vi "Single Axis motor_Z(SubVI).vi"(0 "State=1, I":dbl, 1 "Motor=0, I":i32, 2 "Position=0, I":dbl, 3 "User Input":dbl, 4 "Motor Input":dbl, 5 "Backward":bool, 6 "Forward":bool, 7 "Step diff":dbl, 9 "Motor input_L":refnum<vi>, 11 "User input_L":refnum<vi>, 13 "Step diff_L":refnum<vi>) -> (15 "right":bool, 17 "down":bool, 18 "State Chart":i32(graph), 19 "Motor State":dbl, 20 "State=1, O":dbl, 21 "Motor=0, O":i32, 22 "Position=0, O":dbl, 23 "Real Output":dbl, 24 "Motor Position":dbl, 25 "up":bool, 26 "left":bool, 27 "Moving":bool)   [LabVIEW 2018]
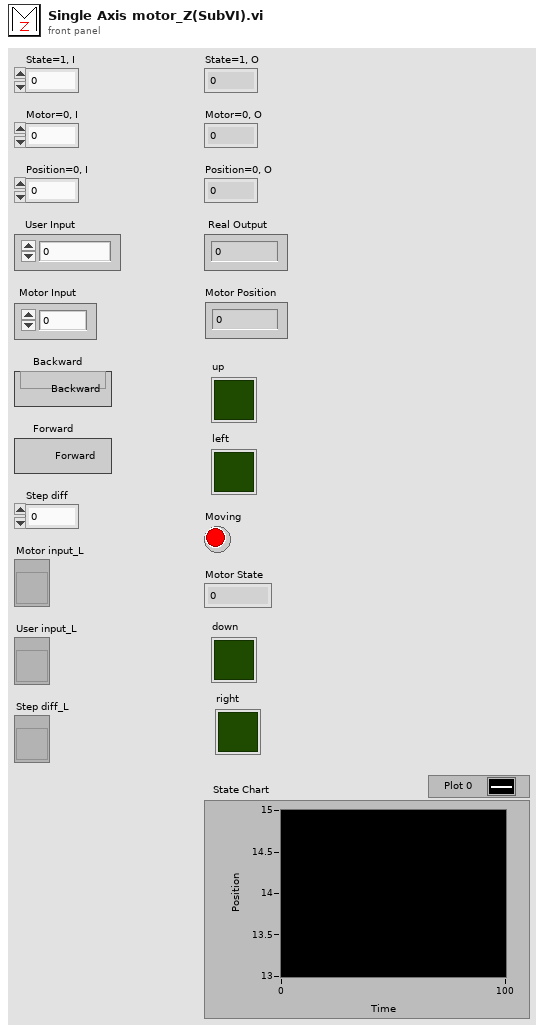
[diagram p1: front panel]
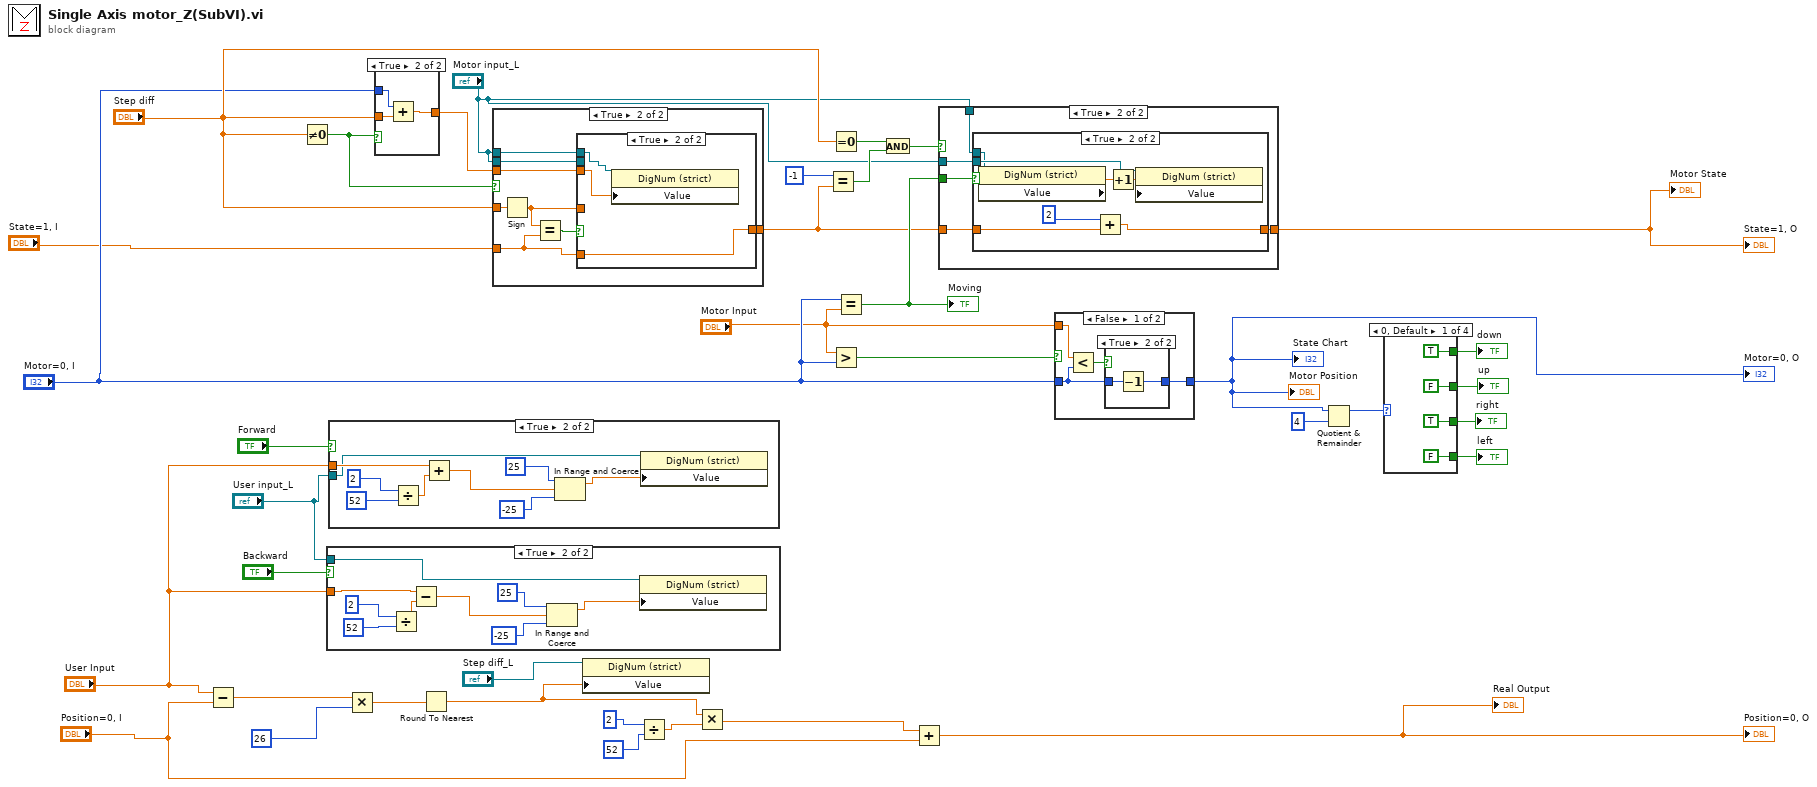
[diagram p0: block diagram]
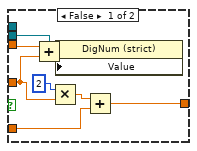
[diagram p7: hidden frame]
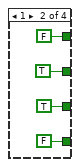
[diagram p8: hidden frame]
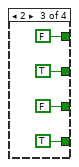
[diagram p9: hidden frame]
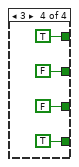
[diagram p10: hidden frame]
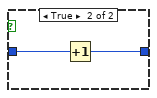
[diagram p12: hidden frame]
diagram:
  n1 = Subtract(x="User Input", y="Position=0, I") -> (x-y=w15:dbl)
  n2 = Not Equal To 0?(x="Step diff") -> (x != 0?=w9:bool)
  n3 = case shown="True" "Backward" {
    tunnel: "User Input" -> [_ w43]
    tunnel: "User input_L" -> [_ w42]
    frame False {
    }
    frame True {
      n4 = Divide(x=2, y=52) -> (x/y=w44:dbl)
      n5 = Subtract(x=w43, y=w44) -> (x-y=w39:dbl)
      n6 = In Range and Coerce(upper limit=25, x=w39, lower limit=-25) -> (coerced(x)=w38:dbl)  [unwired: 1 out]
      n7 = property class="DigNum (strict)"(reference=w42, "Value"=w38) -> ()  [unwired: 1 in, 2 out]
    }
  }
  n8 = case shown="True" "Forward" {
    tunnel: "User Input" -> [_ w52]
    tunnel: "User input_L" -> [_ w51]
    frame False {
    }
    frame True {
      n9 = Divide(x=2, y=52) -> (x/y=w53:dbl)
      n10 = Add(x=w52, y=w53) -> (x+y=w48:dbl)
      n11 = In Range and Coerce(upper limit=25, x=w48, lower limit=-25) -> (coerced(x)=w47:dbl)  [unwired: 1 out]
      n12 = property class="DigNum (strict)"(reference=w51, "Value"=w47) -> ()  [unwired: 1 in, 2 out]
    }
  }
  n13 = Multiply(x=w15, y=26) -> (x*y=w16:dbl)
  n14 = case shown="True" w9 {
    tunnel: "Motor=0, I" -> [_ w59]
    tunnel: "Step diff" -> [w56 w58]
    tunnel: [w56 w57] -> w10
    frame False {
    }
    frame True {
      n15 = Add(x=w59, y=w58) -> (x+y=w57:dbl)
    }
  }
  n16 = Round To Nearest(number=w16) -> (nearest integer value=w20:dbl)
  n17 = case shown="True" w9 {
    tunnel: [w60 w67] -> w26
    tunnel: "State=1, I" -> [w60 w66]
    tunnel: "Step diff" -> [_ w64]
    tunnel: w10 -> [_ w63]
    tunnel: "Motor input_L" -> [_ w62]
    tunnel: "Motor input_L" -> [_ w61]
    frame False {
    }
    frame True {
      n18 = Sign(1:w64) -> (0:w65:dbl)
      n19 = Equal?(x=w65, y=w66) -> (x = y?=w68:bool)
      n20 = case shown="True" w68 {
        tunnel: w65 -> [w70 _]
        tunnel: [w75 w79] -> w67
        tunnel: w66 -> [w73 w79]
        tunnel: w63 -> [w72 w78]
        tunnel: w62 -> [w69 _]
        tunnel: w61 -> [_ w77]
        frame False {
          n21 = Add(x=w72, y=w70) -> (x+y=w74:dbl)
          n22 = Multiply(x=2, y=w70) -> (x*y=w71:dbl)
          n23 = property class="DigNum (strict)"(reference=w69, "Value"=w74) -> ()  [unwired: 1 in, 2 out]
          n24 = Add(x=w71, y=w73) -> (x+y=w75:dbl)
        }
        frame True {
          n25 = property class="DigNum (strict)"(reference=w77, "Value"=w78) -> ()  [unwired: 1 in, 2 out]
        }
      }
    }
  }
  n26 = property class="DigNum (strict)"(reference="Step diff_L", "Value"=w20) -> ()  [unwired: 1 in, 2 out]
  n27 = Divide(x=2, y=52) -> (x/y=w19:dbl)
  n28 = Multiply(x=w20, y=w19) -> (x*y=w6:dbl)
  n29 = Equal?(x=-1, y=w26) -> (x = y?=w25:bool)
  n30 = Equal To 0?(x="Step diff") -> (x = 0?=w24:bool)
  n31 = Greater?(x="Motor Input", y="Motor=0, I") -> (0:w8:bool)
  n32 = Equal?(x="Motor=0, I", y="Motor Input") -> (x = y?=w36:bool)
  "Moving" <- w36
  n33 = And(x=w24, y=w25) -> (x .and. y?=w23:bool)
  n34 = Add(x=w6, y="Position=0, I") -> (x+y=→"Real Output" →"Position=0, O":dbl)
  n35 = case shown="True" w23 {
    tunnel: w26 -> [w80 w84]
    tunnel: [w80 w85] -> w22
    tunnel: w36 -> [_ w83]
    tunnel: "Motor input_L" -> [_ w82]
    tunnel: "Motor input_L" -> [_ w81]
    frame False {
    }
    frame True {
      n36 = case shown="True" w83 {
        tunnel: [w86 w91] -> w85
        tunnel: w84 -> [w86 w92]
        tunnel: w82 -> [_ w88]
        tunnel: w81 -> [_ w87]
        frame False {
        }
        frame True {
          n37 = property class="DigNum (strict)"(reference=w87) -> ("Value"=w89:dbl)  [unwired: 1 in, 2 out]
          n38 = Add(x=2, y=w92) -> (x+y=w91:dbl)
          n39 = Increment(x=w89) -> (x+1=w90:dbl)
          n40 = property class="DigNum (strict)"(reference=w88, "Value"=w90) -> ()  [unwired: 1 in, 2 out]
        }
      }
    }
  }
  "Motor State" <- w22
  "State=1, O" <- w22
  n41 = case shown="False" w8 {
    tunnel: "Motor=0, I" -> [w95 w102]
    tunnel: [w94 w101] -> w21
    tunnel: "Motor Input" -> [w97 _]
    frame False {
      n42 = Less?(x=w97, y=w95) -> (x < y?=w96:bool)
      n43 = case shown="True" w96 {
        tunnel: w95 -> [w98 w100]
        tunnel: [w98 w99] -> w94
        frame False {
        }
        frame True {
          n44 = Decrement(x=w100) -> (x-1=w99:i32)
        }
      }
    }
    frame True {
      n45 = Increment(x=w102) -> (x+1=w101:i32)
    }
  }
  "State Chart" <- w21
  "Motor Position" <- w21
  "Motor=0, O" <- w21
  n46 = Quotient & Remainder(x=w21, y=4) -> (x-y*floor(x/y)=w28:i32)  [unwired: 1 out]
  n47 = case shown="0, Default" w28 {
    tunnel: [FALSE FALSE TRUE TRUE] -> w32
    tunnel: [TRUE TRUE FALSE FALSE] -> w31
    tunnel: [FALSE TRUE TRUE FALSE] -> w30
    tunnel: [TRUE FALSE FALSE TRUE] -> w29
    frame 0, Default {
    }
    frame 1 {
    }
    frame 2 {
    }
    frame 3 {
    }
  }
  "up" <- w30
  "down" <- w29
  "right" <- w31
  "left" <- w32
